vi "LaunchControlPanel.vi"() -> ()   [LabVIEW 2014, in "zsLaunch.lvlib" / "Launcher.lvclass"]
uses:
  Launcher.lvclass
  ControlPanel_lib/Input Operator/ControlPanel.lvclass
  <vilib>/ActorFramework/Actor/Actor.lvclass
panel:
  out "error out":errorcluster caption="错误输出"
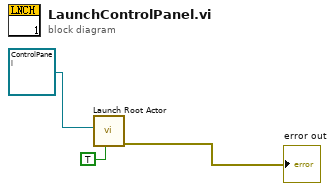
[diagram p0: block diagram]
diagram:
  n1 = call <vilib>:"Launch Root Actor.vi"("Open Actor Core front panel? (F)"=TRUE, "Actor"=refnum<class "ControlPanel.lvclass"> refnum ("ControlPanel.lvlib:ControlPanel.lvclass")) -> ("error out"=→"error out":errorcluster)  [unwired: 8 in, 1 out]
